vi "Read String Channel Properties.vi"(8 "error in (no error)":errorcluster, 10 "String Channel ID":string, 11 "Channel in":refnum<class "Channel.lvclass">) -> (0 "error out":errorcluster, 2 "String Channel":T1, 3 "Channel out":refnum<class "Channel.lvclass">)   [LabVIEW 2026, in "Modbus.lvlib" / "Modbus.lvclass"]
uses:
  Modbus.lvclass
  <vilib>/FlexLogger/SDK/PluginSDK.lvlibp/PEFClasses/SDK/Channel/Channel.lvclass
  Types/String Data.ctl
  Types/Modbus Table.ctl
  Globals/Modbus Strings.vi
  <vilib>/FlexLogger/SDK/PluginSDK.lvlibp/PEFClasses/SDK/Channel/ParameterAccess/Read Enum.vi
  <vilib>/FlexLogger/SDK/PluginSDK.lvlibp/PEFClasses/SDK/Channel/ParameterAccess/Read I32.vi
  <vilib>/FlexLogger/SDK/PluginSDK.lvlibp/PEFClasses/SDK/Channel/Read Valid.vi
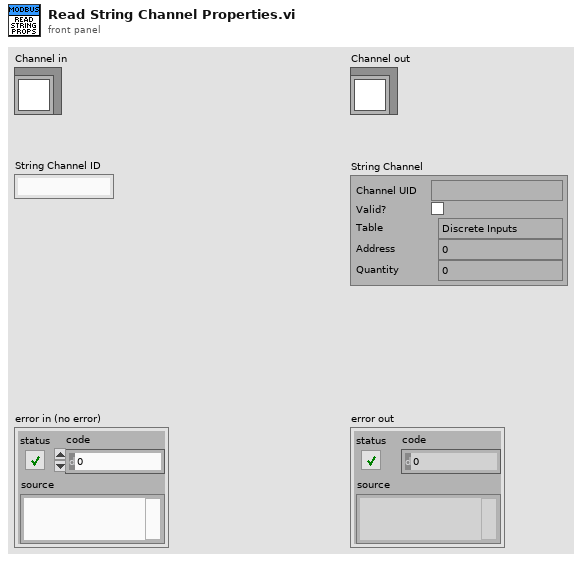
[diagram p1: front panel]
types:
  T1 = typedef "Modbus.lvlib/Modbus.lvclass/String Data.ctl" = cluster{"Channel UID":string, "Valid?":bool, "Table":T2, "Address":i32, "Quantity":u16}
  T2 = typedef "Modbus.lvlib/Modbus.lvclass/Modbus Table.ctl" = enum16{"Discrete Inputs", "Coils", "Input Registers", "Holding Registers"}
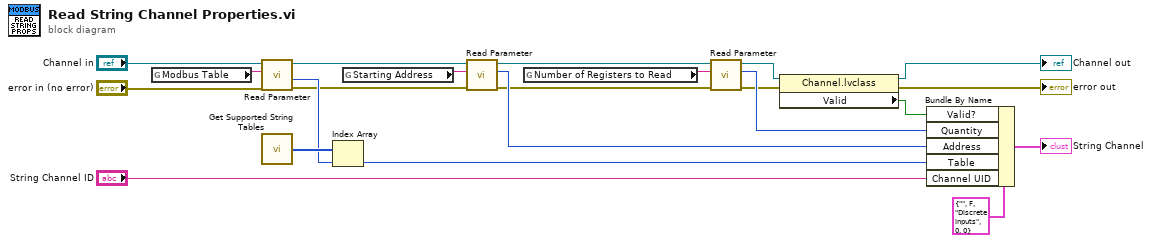
[diagram p0: block diagram]
diagram:
  n1 = global read "Modbus Strings.vi" "Modbus Table"() -> (w15:string)
  n2 = call-poly <vilib>:"Read Parameter.vi"("error in (no error)"="error in (no error)", "Name"=w15, "Channel in"="Channel in") -> ("error out"=w17:errorcluster, "Index"=w19:i32, "Channel out"=w16:refnum<class "Channel.lvclass">)  [unwired: 4 in, 2 out]
  n3 = call "Get Supported String Tables.vi"() -> ("Supported Tables"=w22:T2[])  [unwired: 1 in]
  n4 = Index Array(array=w22, index=w19) -> (element=w20:T2)
  n5 = global read "Modbus Strings.vi" "Starting Address"() -> (w18:string)
  n6 = call-poly <vilib>:"Read Parameter.vi"("error in (no error)"=w17, "Name"=w18, "Channel in"=w16) -> ("error out"=w4:errorcluster, "Value"=w21:i32, "Channel out"=w5:refnum<class "Channel.lvclass">)  [unwired: 5 in, 1 out]
  n7 = global read "Modbus Strings.vi" "Number of Registers to Read"() -> (w6:string)
  n8 = call-poly <vilib>:"Read Parameter.vi"("error in (no error)"=w4, "Name"=w6, "Channel in"=w5) -> ("error out"=w2:errorcluster, "Value"=w3:i32, "Channel out"=w1:refnum<class "Channel.lvclass">)  [unwired: 5 in, 1 out]
  n9 = property class="Channel.lvclass"(reference=w1, error in=w2) -> (reference out=→"Channel out":refnum<class "Channel.lvclass">, error out=→"error out":errorcluster, "Valid"=w10:bool)
  n10 = Bundle By Name(cluster=T1 {"Channel UID"="", "Valid?"=FALSE, "Table"=enum."Discrete Inputs", "Address"=0, "Quantity"=0} ("String Data"), "Valid?"=w10, "Quantity"=w3, "Address"=w21, "Table"=w20, "Channel UID"="String Channel ID") -> (→"String Channel":T1)
